vi "upload.tdms.vi"(8 "error in":errorcluster, 10 "File Path":path, 11 "Nominal Client in":refnum<class "Nominal Client.lvclass">) -> (0 "error out":errorcluster, 3 "Nominal Client out":refnum<class "Nominal Client.lvclass">)   [LabVIEW 2020, in "Nominal Client.lvclass"]
doc: "This VI uploads a specified TDMS file to the Nominal platform. Only channels containing waveform data types are uploaded, ensuring that other unsupported data types are ignored. All properties associated with the waveform channels are preserved and uploaded alongside the data. The VI waits for the Nominal platform to fully ingest the TDMS file before completing its execution, ensuring data integrity and confirmation of successful upload."
uses:
  Nominal Client.lvclass
  <vilib>/dlg_ctls.llb/Space Constant.vi
  catalog.wait_until_multiple_ingest_complete.vi
  Nominal Client.lvclass/Nominal Client.ctl
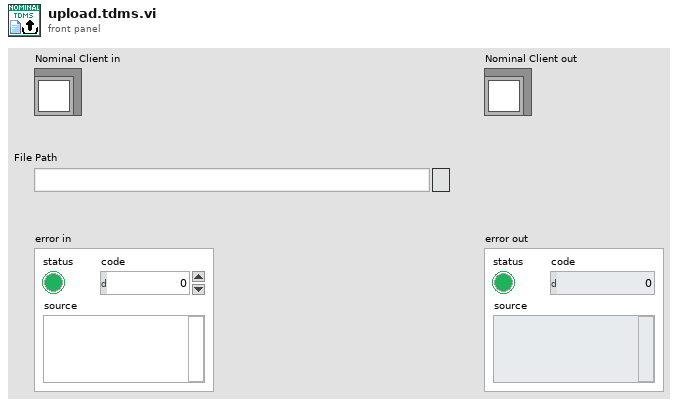
[diagram p1: front panel]
types:
  T1 = enum16{"open", "open or create", "create or replace", "create", "open (read-only)"}
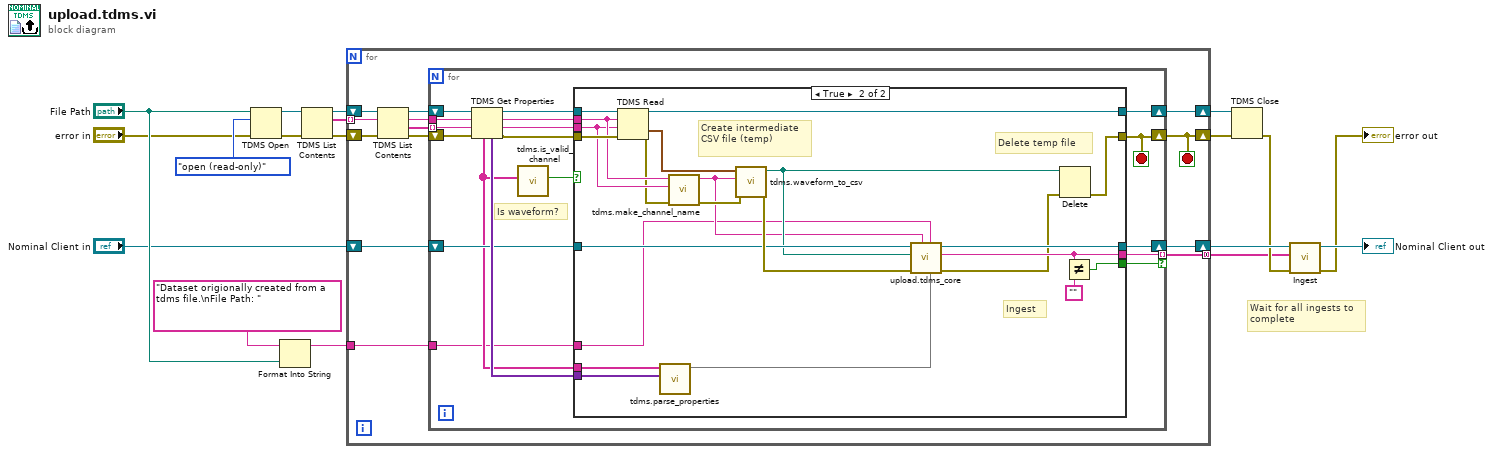
[diagram p0: block diagram]
diagram:
  # "Wait for all ingests to complete"
  n1 = TDMS Open(8:"error in", 10:T1."open (read-only)" ("operation (0:open)"), 11:"File Path") -> (0:w17:errorcluster, 3:w18:refnum<k34>)  [unwired: 4 in]
  n2 = Format Into String(initial string="Dataset origionally created from a tdms file.\nFile Path: ", "File Path") -> (resulting string=w7:string)  [unwired: 2 in, 1 out]
  n3 = TDMS List Contents(4:w17, 7:w18) -> (0:w4:errorcluster, 2:w13:string[], 3:w16:refnum<k34>)  [unwired: 1 in, 1 out]
  n4 = for {
    shift-right: [w24] -> w14
    shift-left: w16 -> [w31]
    shift-right: [w19] -> w15
    shift-left: w4 -> [w30]
    tunnel: w13 -> [w29] mode=indexing
    shift-right: [w23] -> w12
    shift-left: "Nominal Client in" -> [w22]
    tunnel: [w21] -> w6 mode=concatenating
    tunnel: w7 -> [w20]
    stop <- w19 stop-if-true
    n5 = TDMS List Contents(4:w30, 6:w29, 7:w31) -> (0:w25:errorcluster, 1:w26:string[], 2:w27:string, 3:w28:refnum<k34>)
    n6 = for {
      tunnel: w27 -> [w46]
      tunnel: w26 -> [w45] mode=indexing
      shift-right: [w32] -> w19
      shift-left: w25 -> [w48]
      shift-right: [w42] -> w24
      shift-left: w28 -> [w49]
      shift-right: [w39] -> w23
      shift-left: w22 -> [w38]
      tunnel: [w35] -> w21 mode=indexing if=w34
      tunnel: w20 -> [w33]
      stop <- w32 stop-if-true
      # "Is waveform?"
      n7 = TDMS Get Properties(8:w48, 9:w45, 10:w46, 11:w49) -> (0:w43:errorcluster, 1:w40:string, 2:w41:string, 3:w44:refnum<k34>, 4:w47:variant[], 6:w37:string[])  [unwired: 2 in]
      n8 = call "tdms.is_valid_channel.vi"("TDMS Property Names"=w37) -> ("Valid Channel"=w36:bool)  [unwired: 10 in]
      n9 = case shown="True" w36 {
        tunnel: w47 -> [_ w67]
        tunnel: w37 -> [_ w68]
        tunnel: w44 -> [w52 w74]
        tunnel: w43 -> [w51 w73]
        tunnel: [w52 w72] -> w42
        tunnel: [w51 w62] -> w32
        tunnel: w41 -> [_ w70]
        tunnel: w40 -> [_ w69]
        tunnel: [w50 w60] -> w39
        tunnel: w38 -> [w50 w57]
        tunnel: [_ w61] -> w35
        tunnel: [_ w65] -> w34
        tunnel: w33 -> [_ w54]
        frame False {
        }
        frame True {
          # "Ingest"
          # "Delete temp file"
          # "Create intermediate CSV file (temp)"
          n10 = TDMS Read(0:w74, 5:w70, 7:w69, 11:w73) -> (4:w72:refnum<k34>, 10:w71:waveform(dbl), 15:w63:errorcluster)  [unwired: 4 in, 3 out]
          n11 = call "tdms.parse_properties.vi"("Property Values"=w67, "Property Names"=w68) -> ("Property Map"=w53:map{string, string})  [unwired: 9 in]
          n12 = call "tdms.make_channel_name.vi"("error in"=w63, "Channel Name"=w69, "Group Name"=w70) -> ("error out"=w66:errorcluster, "channel name"=w55:string)  [unwired: 7 in]
          n13 = call "tdms.waveform_to_csv.vi"("error in"=w66, "Formatted Channel Name"=w55, "Waveform"=w71) -> ("error out"=w58:errorcluster, "new csv filepath"=w56:path)  [unwired: 7 in]
          n14 = call "upload.tdms_core.vi"("Properties"=w53, "Description"=w54, "Name"=w55, "error in"=w58, "File Path"=w56, "Nominal Client in"=w57) -> ("error out"=w59:errorcluster, "datasetRID"=w61:string, "Nominal Client out"=w60:refnum<class "Nominal Client.lvclass">)  [unwired: 3 in]
          n15 = Delete(path (use dialog)=w56, error in=w59) -> (error out=w62:errorcluster)  [unwired: 3 in, 2 out]
          n16 = Not Equal?(x=w61, y="") -> (x != y?=w65:bool)
        }
      }
    }
  }
  n17 = TDMS Close(8:w15, 11:w14) -> (0:w11:errorcluster)  [unwired: 1 out]
  n18 = call-poly "Ingest.vi"("error in"=w11, "datasetRid"=w6, "Nominal Client"=w12) -> ("error out"=→"error out":errorcluster, "Nominal Client out"=→"Nominal Client out":refnum<class "Nominal Client.lvclass">)  [unwired: 7 in]
